vi "Wait for Motor Complete.vi"(8 "error in (no error)":errorcluster, 11 "VISA Refnum in":refnum<visa-resource-name>) -> (0 "error out":errorcluster)   [LabVIEW 2023, in "Turn Table and Mast.lvlib" / "CO3000.lvclass"]
uses:
  CO3000.lvclass
  CO3000.lvclass/CO3000.ctl
panel:
  out "Numeric":i32
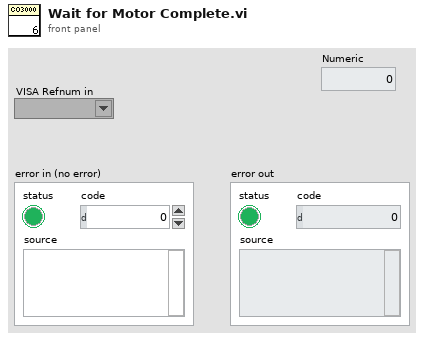
[diagram p1: front panel]
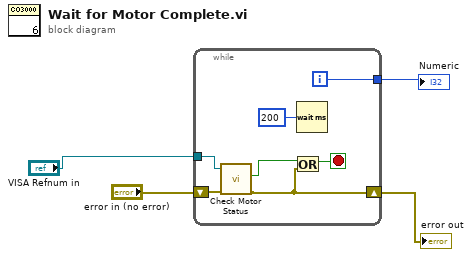
[diagram p0: block diagram]
diagram:
  n1 = while {
    shift-right: [w8] -> w3
    shift-left: "error in (no error)" -> [w9]
    tunnel: "VISA Refnum in" -> [w7]
    tunnel: [w5] -> w1
    i -> [w5]
    stop <- w10 stop-if-true
    n2 = call "Check Motor Status.vi"("error in (no error)"=w9, "VISA Refnum in"=w7) -> ("error out"=w8:errorcluster, "Motor Stop?"=w6:bool)  [unwired: 7 in, 1 out]
    n3 = Or(x=w6, y=w8) -> (x .or. y?=w10:bool)
    n4 = Wait (ms)(milliseconds to wait=u32 200 ("대기 시간 (ms)")) -> ()  [unwired: 1 out]
  }
  "error out" <- w3
  "Numeric" <- w1
